vi "subGetItemInfosFromProjectFile.vi"(8 "error in (no error)":errorcluster, 11 "SolutionBuilder in":refnum<class "SolutionBuilder.lvclass">) -> (0 "error out":errorcluster, 3 "SolutionBuilder out":refnum<class "SolutionBuilder.lvclass">)   [LabVIEW 2019, in "SolutionBuilder.lvlib" / "SolutionBuilder.lvclass"]
uses:
  SolutionBuilder.lvclass
  SolutionBuilder.lvclass/SolutionBuilder.ctl
  ProjectItem/ProjectItem.lvclass
  ProjectItem/ProjectItem.lvclass/ProjectItem.ctl
  1413a22b-f5ab-415a-875b-e08797a96725.vi
  <vilib>/xml/Load XML File.vi
  <vilib>/xml/Close Reference(Node).vi
  <vilib>/xml/NI_XML.lvlib
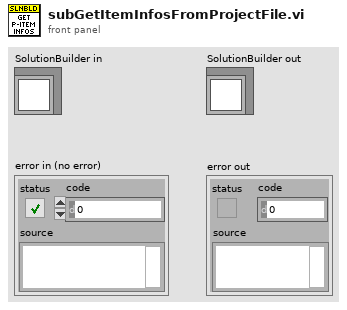
[diagram p1: front panel]
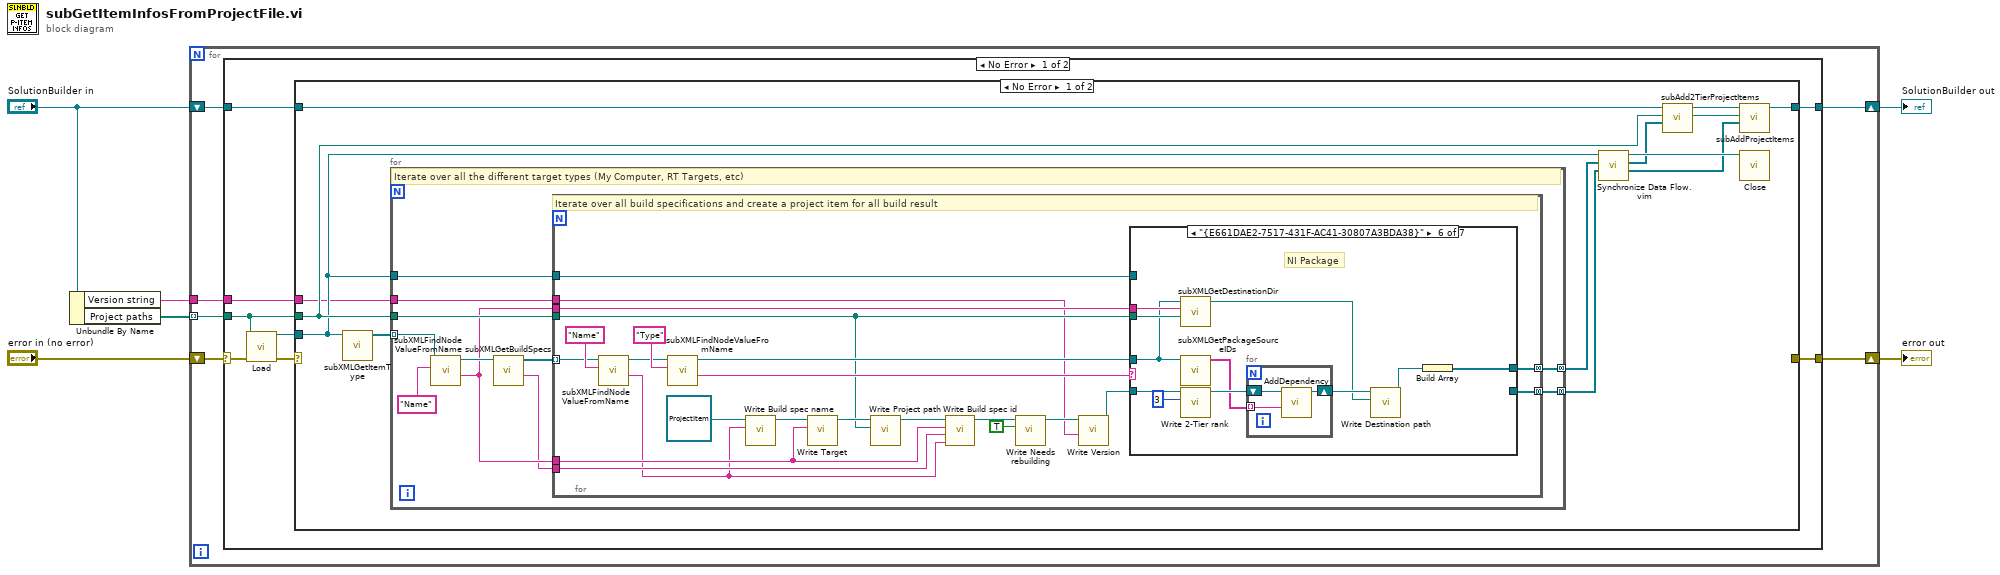
[diagram p0: block diagram]
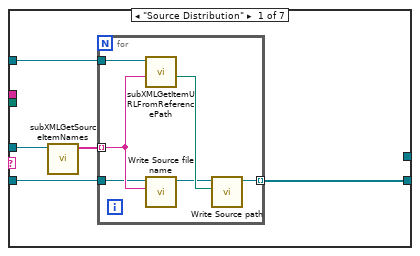
[diagram p2: hidden frame]
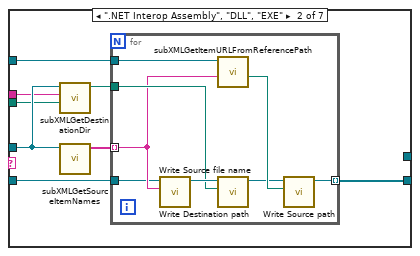
[diagram p3: hidden frame]
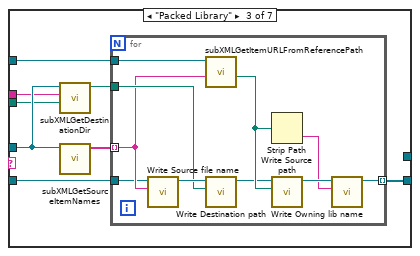
[diagram p4: hidden frame]
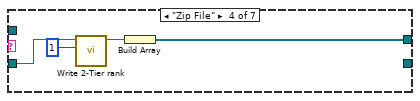
[diagram p5: hidden frame]
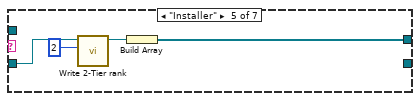
[diagram p6: hidden frame]
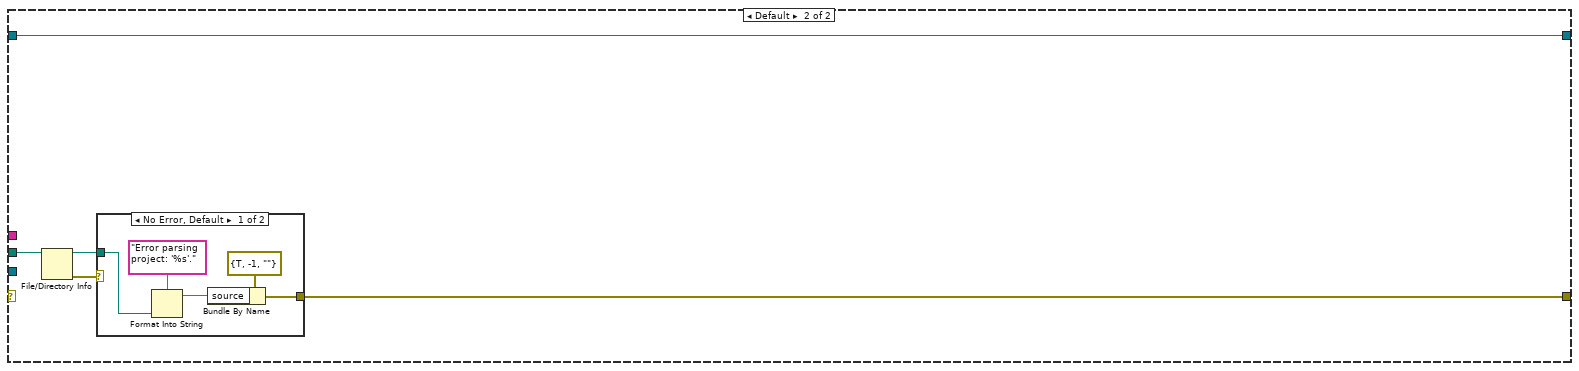
[diagram p8: hidden frame]
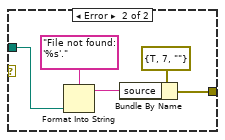
[diagram p9: hidden frame]
diagram:
  n1 = Unbundle By Name("SolutionBuilder in") -> ("Version string"=w1:string, "Project paths"=w6:path[])
  n2 = for {
    tunnel: w6 -> [w11] mode=indexing
    shift-right: [w10] -> w4
    shift-left: "SolutionBuilder in" -> [w12]
    shift-right: [w9] -> w3
    shift-left: "error in (no error)" -> [w8]
    tunnel: w1 -> [w7]
    n3 = case shown="No Error" w8 {
      selector: w8 -> [w14 w150]
      tunnel: w12 -> [w19 w149]
      tunnel: w11 -> [w18 _]
      tunnel: [w17 w149] -> w10
      tunnel: [w15 w150] -> w9
      tunnel: w7 -> [w13 _]
      frame No Error {
        n4 = call-poly <vilib>:"Load.vi"("path to XML document"=w18, "error in (no error)"=w14) -> ("DOM document out"=w20:refnum<k20>, "error out"=w16:errorcluster)  [unwired: 11 in, 1 out]
        n5 = case shown="No Error" w16 {
          tunnel: w20 -> [w25 _]
          tunnel: w19 -> [w29 w138]
          tunnel: w18 -> [w27 w135]
          tunnel: [w32 w138] -> w17
          tunnel: [_ w137] -> w15
          tunnel: w13 -> [w21 _]
          frame No Error {
            n6 = call "subXMLGetItemType.vi"("Refnum in"=w25) -> ("Nodes"=w24:refnum<k20>[])  [unwired: 10 in]
            n7 = for {
              tunnel: [w42] -> w23 mode=concatenating
              tunnel: [w41] -> w22 mode=concatenating
              tunnel: w27 -> [w40]
              tunnel: w25 -> [w39]
              tunnel: w24 -> [w37] mode=indexing
              tunnel: w21 -> [w33]
              # "Iterate over all the different target types (My Computer, RT Targets, etc)"
              n8 = call "subXMLFindNodeValueFromName.vi"("Property name"="Name", "Refnum in"=w37) -> ("Value"=w35:string, "Refnum out"=w36:refnum<k20>)  [unwired: 7 in, 1 out]
              n9 = call "subXMLGetBuildSpecs.vi"("Refnum in"=w36) -> ("Buid spec section"=w34:string, "Nodes"=w43:refnum<k20>[])  [unwired: 9 in]
              n10 = for {
                tunnel: w43 -> [w61] mode=indexing
                tunnel: w40 -> [w51]
                tunnel: [w60] -> w42 mode=concatenating
                tunnel: w39 -> [w59]
                tunnel: [w58] -> w41 mode=concatenating
                tunnel: w35 -> [w48]
                tunnel: w35 -> [w57]
                tunnel: w34 -> [w52]
                tunnel: w33 -> [w44]
                # "Iterate over all build specifications and create a project item for all build result"
                n11 = call "subXMLFindNodeValueFromName.vi"("Property name"="Name", "Refnum in"=w61) -> ("Value"=w47:string, "Refnum out"=w62:refnum<k20>)  [unwired: 7 in, 1 out]
                n12 = call "subXMLFindNodeValueFromName.vi"("Property name"="Type", "Refnum in"=w62) -> ("Value"=w65:string, "Refnum out"=w64:refnum<k20>)  [unwired: 7 in, 1 out]
                n13 = call "Write Build spec name.vi"("Build spec name"=w47, "ProjectItem in"=refnum<class "ProjectItem.lvclass"> refnum ("SolutionBuilder.lvlib:ProjectItem.lvclass")) -> ("ProjectItem out"=w55:refnum<class "ProjectItem.lvclass">)  [unwired: 9 in]
                n14 = call "Write Target.vi"("Target"=w48, "ProjectItem in"=w55) -> ("ProjectItem out"=w56:refnum<class "ProjectItem.lvclass">)  [unwired: 9 in]
                n15 = call "Write Project path.vi"("Project path"=w51, "ProjectItem in"=w56) -> ("ProjectItem out"=w53:refnum<class "ProjectItem.lvclass">)  [unwired: 9 in]
                n16 = call-dynamic "Write Build spec id.vi"("Build spec name"=w47, "Buid spec section"=w52, "Target"=w48, "ProjectItem in"=w53) -> ("ProjectItem out"=w49:refnum<class "ProjectItem.lvclass">)  [unwired: 7 in]
                n17 = call "Write Needs rebuilding.vi"("Needs rebuilding"=TRUE, "ProjectItem in"=w49) -> ("ProjectItem out"=w46:refnum<class "ProjectItem.lvclass">)  [unwired: 9 in]
                n18 = call "Write Version.vi"("Version string"=w44, "ProjectItem in"=w46) -> ("ProjectItem out"=w45:refnum<class "ProjectItem.lvclass">)  [unwired: 9 in]
                n19 = case shown="\"{E661DAE2-7517-431F-AC41-30807A3BDA38}\"" w65 {
                  tunnel: w64 -> [w71 w83 w99 _ _ w120 _]
                  tunnel: [w69 w84 w100 _ _ _ _] -> w60
                  tunnel: w59 -> [w68 w81 w97 _ _ _ _]
                  tunnel: [_ _ _ w113 w117 w129 _] -> w58
                  tunnel: w57 -> [_ w80 w96 _ _ w125 _]
                  tunnel: w45 -> [w67 w79 w95 w112 w116 w128 _]
                  tunnel: w51 -> [_ w78 w94 _ _ w124 _]
                  frame "Source Distribution" {
                    n20 = call "subXMLGetSourceItemNames.vi"("Refnum in"=w71) -> ("Names"=w70:string[])  [unwired: 10 in]
                    n21 = for {
                      tunnel: w70 -> [w76] mode=indexing
                      tunnel: [w74] -> w69 mode=indexing
                      tunnel: w68 -> [w77]
                      tunnel: w67 -> [w72]
                      n22 = call "subXMLGetItemURLFromReferencePath.vi"("Reference path"=w76, "Root ref"=w77) -> ("Path"=w75:path)  [unwired: 7 in, 2 out]
                      n23 = call "Write Source file name.vi"("Source file name"=w76, "ProjectItem in"=w72) -> ("ProjectItem out"=w73:refnum<class "ProjectItem.lvclass">)  [unwired: 9 in]
                      n24 = call "Write Source path.vi"("Source path"=w75, "ProjectItem in"=w73) -> ("ProjectItem out"=w74:refnum<class "ProjectItem.lvclass">)  [unwired: 9 in]
                    }
                  }
                  frame ".NET Interop Assembly", "DLL", "EXE" {
                    n25 = call "subXMLGetDestinationDir.vi"("Project path"=w78, "TargetName"=w80, "Refnum in"=w83) -> ("Path"=w82:path)  [unwired: 7 in, 1 out]
                    n26 = call "subXMLGetSourceItemNames.vi"("Refnum in"=w83) -> ("Names"=w85:string[])  [unwired: 10 in]
                    n27 = for {
                      tunnel: w85 -> [w90] mode=indexing
                      tunnel: [w88] -> w84 mode=indexing
                      tunnel: w82 -> [w92]
                      tunnel: w81 -> [w91]
                      tunnel: w79 -> [w87]
                      n28 = call "Write Source file name.vi"("Source file name"=w90, "ProjectItem in"=w87) -> ("ProjectItem out"=w93:refnum<class "ProjectItem.lvclass">)  [unwired: 9 in]
                      n29 = call "subXMLGetItemURLFromReferencePath.vi"("Reference path"=w90, "Root ref"=w91) -> ("Path"=w89:path)  [unwired: 7 in, 2 out]
                      n30 = call "Write Destination path.vi"("Destination path"=w92, "ProjectItem in"=w93) -> ("ProjectItem out"=w86:refnum<class "ProjectItem.lvclass">)  [unwired: 9 in]
                      n31 = call "Write Source path.vi"("Source path"=w89, "ProjectItem in"=w86) -> ("ProjectItem out"=w88:refnum<class "ProjectItem.lvclass">)  [unwired: 9 in]
                    }
                  }
                  frame "Packed Library" {
                    n32 = call "subXMLGetDestinationDir.vi"("Project path"=w94, "TargetName"=w96, "Refnum in"=w99) -> ("Path"=w98:path)  [unwired: 7 in, 1 out]
                    n33 = call "subXMLGetSourceItemNames.vi"("Refnum in"=w99) -> ("Names"=w101:string[])  [unwired: 10 in]
                    n34 = for {
                      tunnel: w101 -> [w108] mode=indexing
                      tunnel: [w106] -> w100 mode=indexing
                      tunnel: w98 -> [w110]
                      tunnel: w97 -> [w109]
                      tunnel: w95 -> [w102]
                      n35 = call "Write Source file name.vi"("Source file name"=w108, "ProjectItem in"=w102) -> ("ProjectItem out"=w111:refnum<class "ProjectItem.lvclass">)  [unwired: 9 in]
                      n36 = call "subXMLGetItemURLFromReferencePath.vi"("Reference path"=w108, "Root ref"=w109) -> ("Path"=w105:path)  [unwired: 7 in, 2 out]
                      n37 = call "Write Destination path.vi"("Destination path"=w110, "ProjectItem in"=w111) -> ("ProjectItem out"=w103:refnum<class "ProjectItem.lvclass">)  [unwired: 9 in]
                      n38 = Strip Path(path=w105) -> (name=w104:string)  [unwired: 1 out]
                      n39 = call "Write Source path.vi"("Source path"=w105, "ProjectItem in"=w103) -> ("ProjectItem out"=w107:refnum<class "ProjectItem.lvclass">)  [unwired: 9 in]
                      n40 = call "Write Owning lib name.vi"("Owning lib name"=w104, "ProjectItem in"=w107) -> ("ProjectItem out"=w106:refnum<class "ProjectItem.lvclass">)  [unwired: 9 in]
                    }
                  }
                  frame "Zip File" {
                    n41 = call "Write 2-Tier rank.vi"("2-Tier rank"=u8 1, "ProjectItem in"=w112) -> ("ProjectItem out"=w115:refnum<class "ProjectItem.lvclass">)  [unwired: 9 in]
                    n42 = Build Array(w115) -> (w113:refnum<class "ProjectItem.lvclass">[])
                  }
                  frame "Installer" {
                    n43 = call "Write 2-Tier rank.vi"("2-Tier rank"=u8 2, "ProjectItem in"=w116) -> ("ProjectItem out"=w119:refnum<class "ProjectItem.lvclass">)  [unwired: 9 in]
                    n44 = Build Array(w119) -> (w117:refnum<class "ProjectItem.lvclass">[])
                  }
                  frame "{E661DAE2-7517-431F-AC41-30807A3BDA38}" {
                    # "NI Package"
                    n45 = call "subXMLGetDestinationDir.vi"("Project path"=w124, "TargetName"=w125, "Refnum in"=w120) -> ("Path"=w121:path)  [unwired: 7 in, 1 out]
                    n46 = call "subXMLGetPackageSourceIDs.vi"("Refnum in"=w120) -> ("IDs"=w126:string[])  [unwired: 10 in]
                    n47 = call "Write 2-Tier rank.vi"("2-Tier rank"=u8 3, "ProjectItem in"=w128) -> ("ProjectItem out"=w127:refnum<class "ProjectItem.lvclass">)  [unwired: 9 in]
                    n48 = for {
                      shift-right: [w132] -> w123
                      shift-left: w127 -> [w133]
                      tunnel: w126 -> [w131] mode=indexing
                      n49 = call "AddDependency.vi"("Dependency"=w131, "ProjectItem in"=w133) -> ("ProjectItem out"=w132:refnum<class "ProjectItem.lvclass">)  [unwired: 8 in, 1 out]
                    }
                    n50 = call "Write Destination path.vi"("Destination path"=w121, "ProjectItem in"=w123) -> ("ProjectItem out"=w122:refnum<class "ProjectItem.lvclass">)  [unwired: 9 in]
                    n51 = Build Array(w122) -> (w129:refnum<class "ProjectItem.lvclass">[])
                  }
                  frame Default {
                  }
                }
              }
            }
            n52 = call "Synchronize Data Flow.vim"("input 3"=w23, "input 2"=w22, "input 1"=w25) -> ("output 3"=w30:refnum<class "ProjectItem.lvclass">[], "output 2"=w26:refnum<class "ProjectItem.lvclass">[], "output 1"=w31:refnum<k20>)  [unwired: 1 in, 1 out]
            n53 = call "subAdd2TierProjectItems.vi"("ProjectItems"=w26, "Owning project"=w27, "SolutionBuilder in"=w29) -> ("SolutionBuilder out"=w28:refnum<class "SolutionBuilder.lvclass">)  [unwired: 7 in, 1 out]
            n54 = call "subAddProjectItems.vi"("ProjectItems"=w30, "Owning project"=w27, "SolutionBuilder in"=w28) -> ("SolutionBuilder out"=w32:refnum<class "SolutionBuilder.lvclass">)  [unwired: 7 in, 1 out]
            n55 = call-poly <vilib>:"Close.vi"("node"=w31) -> ()  [unwired: 8 in, 1 out]
          }
          frame Default {
            n56 = File/Directory Info(path=w135) -> (path out=w136:path, error out=w134:errorcluster)  [unwired: 1 in, 5 out]
            n57 = case shown="No Error, Default" w134 {
              tunnel: [w140 w145] -> w137
              tunnel: w136 -> [w139 w144]
              frame No Error {
                n58 = Format Into String(format string="Error parsing project: '%s'.", w139) -> (resulting string=w142:string)  [unwired: 2 in, 1 out]
                n59 = Bundle By Name(cluster=errorcluster {"status"=TRUE, "code"=-1, "source"=""} ("t"), "source"=w142) -> (w140:errorcluster)
              }
              frame Error {
                n60 = Format Into String(format string="File not found: '%s'.", w144) -> (resulting string=w147:string)  [unwired: 2 in, 1 out]
                n61 = Bundle By Name(cluster=errorcluster {"status"=TRUE, "code"=7, "source"=""} ("t"), "source"=w147) -> (w145:errorcluster)
              }
            }
          }
        }
      }
      frame Error {
      }
    }
  }
  "SolutionBuilder out" <- w4
  "error out" <- w3
